vi "ActiveObject_QueueQueue_StartProcess_OnePerClass.vi"(0 "reference in":refnum<class>, 3 "ms timeout (-1)":i32=-1, 5 "Error In":errorcluster) -> (14 "reference out":refnum<class>, 19 "Error Out":errorcluster)   [LabVIEW 2020]
doc: "Looks up an existing object matching object name or creates a new object and returns a refnum you can use when calling other class methods.\n\nObjects created with this VI should be destroyed using this class Delete VI."
panel:
  out "timed out":bool
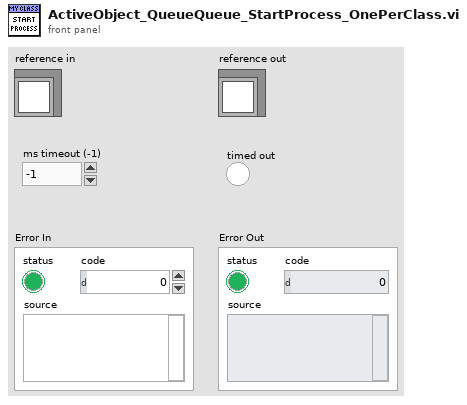
[diagram p1: front panel]
types:
  T1 = enum16{"ReadRepository", "CreateNew", "CreateOrLookUpExisting", "ReadRepositoryAndDestroy"}
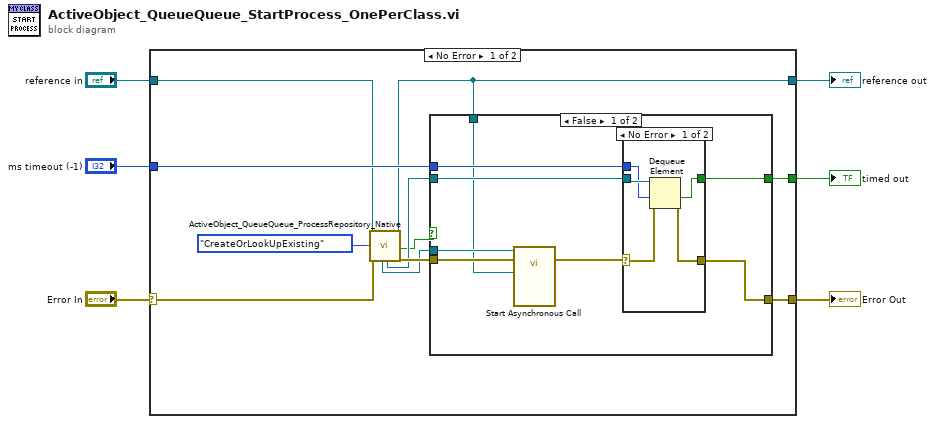
[diagram p0: block diagram]
diagram:
  n1 = case shown="No Error" "Error In" {
    selector: "Error In" -> [w14 w33]
    tunnel: [w15 w33] -> w5
    tunnel: [w10 w34] -> w3
    tunnel: "reference in" -> [w8 w34]
    tunnel: "ms timeout (-1)" -> [w17 _]
    tunnel: [w16 _] -> w1
    frame No Error {
      n2 = call "ActiveObject_QueueQueue_ProcessRepository_Native.vi"("reference in"=w8, "Action(ReadRepository)"=T1."CreateOrLookUpExisting", "Error In"=w14) -> ("ProcessViRef"=w12:refnum<vi>, "ProcessSyncQueue"=w11:refnum<queue>, "reference out"=w10:refnum<class>, "ProcessAlreadyStarted"=w9:bool, "Error Out"=w13:errorcluster)  [unwired: 10 in, 2 out]
      n3 = case shown="False" w9 {
        tunnel: w17 -> [w25 _]
        tunnel: [w24 _] -> w16
        tunnel: [w23 w32] -> w15
        tunnel: w13 -> [w20 w32]
        tunnel: w12 -> [w21 _]
        tunnel: w11 -> [w22 _]
        tunnel: w10 -> [w19 _]
        frame False {
          n4 = call-by-ref "Start Asynchronous Call"(reference=w21, error in=w20, "reference in"=w19) -> (error out=w18:errorcluster)  [unwired: 17 in, 3 out]
          n5 = case shown="No Error" w18 {
            tunnel: w22 -> [w30 _]
            tunnel: w25 -> [w29 _]
            tunnel: [w28 _] -> w24
            selector: w18 -> [w27 w31]
            tunnel: [w26 w31] -> w23
            frame No Error {
              n6 = Dequeue Element(queue=w30, timeout in ms (-1)=w29, error in (no error)=w27) -> (timed out?=w28:bool, error out=w26:errorcluster)  [unwired: 2 out]
            }
            frame Error {
            }
          }
        }
        frame True {
          # "Process Already started.\nThis option will only be used togeather with the\naction: \"CreateOrLookUpExisting\""
        }
      }
    }
    frame Error {
    }
  }
  "Error Out" <- w5
  "reference out" <- w3
  "timed out" <- w1
